vi "DriverStation Game Data.vi"() -> (3 "Game Specific Data":string)   [LabVIEW 2023, in "MrcLib.lvlib"]
doc: "Returns game specific data from the FMS (Field Management System) or DS."
uses:
  <vilib>/MRC/MrcLib.lvlib
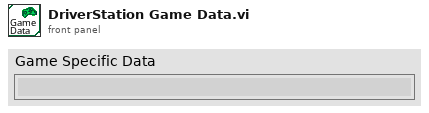
[diagram p1: front panel]
types:
  T1 = typedef "MrcLib.lvlib/MRC_ControlData.ctl" = cluster{"controlFlags":u32, "matchTime":u16, "currentOpMode":u64, "gameDataLength":u8, "game data":T2}
  T2 = typedef "MRC Str64.ctl" = cluster{"[0]":u8, "[1]":u8, "[2]":u8, "[3]":u8, "[4]":u8, "[5]":u8, "[6]":u8, "[7]":u8, "[8]":u8, "[9]":u8, "[10]":u8, "[11]":u8, "[12]":u8, "[13]":u8, "[14]":u8, "[15]":u8, "[16]":u8, "[17]":u8, "[18]":u8, "[19]":u8, "[20]":u8, "[21]":u8, "[22]":u8, "[23]":u8, "[24]":u8, "[25]":u8, "[26]":u8, "[27]":u8, "[28]":u8, "[29]":u8, "[30]":u8, "[31]":u8, "[32]":u8, "[33]":u8, "[34]":u8, "[35]":u8, "[36]":u8, "[37]":u8, "[38]":u8, "[39]":u8, "[40]":u8, "[41]":u8, "[42]":u8, "[43]":u8, "[44]":u8, "[45]":u8, "[46]":u8, "[47]":u8, "[48]":u8, "[49]":u8, "[50]":u8, "[51]":u8, "[52]":u8, "[53]":u8, "[54]":u8, "[55]":u8, "[56]":u8, "[57]":u8, "[58]":u8, "[59]":u8, "[60]":u8, "[61]":u8, "[62]":u8, "[63]":u8}
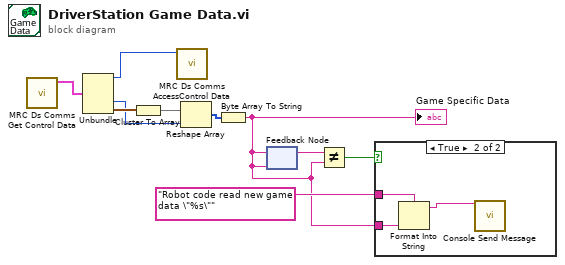
[diagram p0: block diagram]
diagram:
  n1 = call <vilib>:"MRC Ds Comms Get Control Data.vi"() -> ("data out"=w7:T1)  [unwired: 10 in, 1 out]
  n2 = Unbundle(w7) -> ("controlFlags"=w1:u32, "gameDataLength"=w3:u8, "game data"=w4:T2)  [unwired: 2 out]
  n3 = Cluster To Array(cluster=w4) -> (array=w6:u8[])
  n4 = call <vilib>:"MRC Ds Comms AccessControl Data.vi"("controlFlag"=w1) -> ()  [unwired: 7 in, 4 out]
  n5 = Reshape Array(w6, w3) -> (w5:u8[])
  n6 = Byte Array To String(unsigned byte array=w5) -> (string=w2:string)
  "Game Specific Data" <- w2
  n7 = feedback #1(w2) -> (w10:string)
  n8 = feedback-in #1(w2) -> ()
  n9 = Not Equal?(x=w10, y=w2) -> (x != y?=w9:bool)
  n10 = case shown="True" w9 {
    tunnel: "Robot code read new game data \"%s\"" ("Message") -> [_ w13]
    tunnel: w2 -> [_ w12]
    frame False {
    }
    frame True {
      n11 = Format Into String(format string=w13, w12) -> (resulting string=w11:string)  [unwired: 2 in, 1 out]
      n12 = call <vilib>:"Console Send Message.vi"("Message"=w11) -> ()  [unwired: 14 in, 1 out]
    }
  }
